vi "SubTask2.vi"   [LabVIEW 2016]
uses:
  <vilib>/NXT/Block Support/NXT_InputPort.ctl
  <vilib>/NXT/Block Support/NXT_OutputPort.ctl
  <vilib>/NXT/Dual Mode Library/Sensors/EV3_Ultrasonic_CM.vi
  <vilib>/NXT/NXTIO Xnodes/NXTIONodeSubVIs/NXTStopMotors.vi
  <vilib>/NXT/NXTIO Xnodes/NXTIONodeSubVIs/NXTMoveMotors.vi
  <vilib>/NXT/NXTIO Xnodes/AddressXNode/NXTIOAddress.xnode
  PMR_081.lvrbt
  <vilib>/NXT/Subs/LVHSConnector.ctl
  <vilib>/NXT/NXTIO Xnodes/NXTIOXNode/NXTIO.xnode
  <vilib>/NXT/LegoClasses/BrickReference/BrickReference.lvclass
types:
  T1 = typedef "NXT_InputPort.ctl" = u32
  T2 = typedef "NXT_OutputPort.ctl" = u8
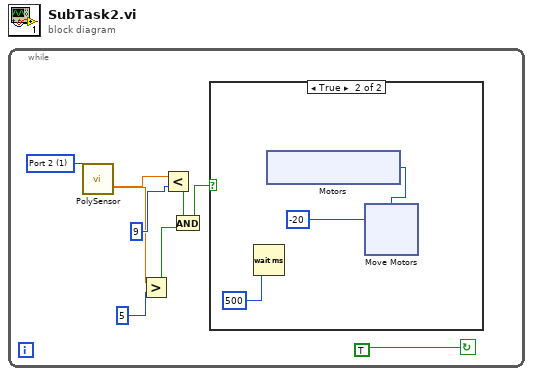
[diagram p0: block diagram]
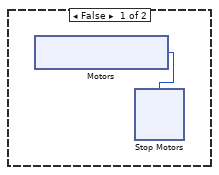
[diagram p2: hidden frame]
diagram:
  n1 = while {
    stop <- TRUE continue-if-true
    w7 = T1 1 items=["Port 1", "Port 2", "Port 3", "Port 4"] ("Port (Port 4)")
    n2 = call-poly <vilib>:"PolySensor.vi"("Port (Port 1)"=w7) -> ("Centimeters"=w4:sgl)  [unwired: 2 in, 1 out]
    n3 = Greater?(x=w4, y=i16 5 ("Distance (cm)")) -> (0:w3:bool)
    n4 = Less?(x=w4, y=i16 9 ("Distance (cm)")) -> (x < y?=w2:bool)
    n5 = And(x=w2, y=w3) -> (x .and. y?=w1:bool)
    n6 = case shown="True" w1 {
      frame False {
        n7 = xnode "Motors"() -> ("Motor"=w9:T2)
        n8 = xnode "Stop Motors"("Motors"=w9) -> ()  [unwired: 1 in, 1 out]
      }
      frame True {
        n9 = Wait (ms)(milliseconds to wait=500) -> ()  [unwired: 1 out]
        n10 = xnode "Motors"() -> ("Motor"=w18:T2)
        n11 = xnode "Move Motors"("Power/Speed 1"=-20, "Motors"=w18) -> ()  [unwired: 1 in, 1 out]
      }
    }
  }
